vi "Read_from_Config_File.vi"(11 "Error In":errorcluster) -> (4 "Debug":bool, 15 "Error Out":errorcluster)   [LabVIEW 2026, in "Core.lvlib"]
doc: "Reads application settings from the configuration file and returns the configured status."
uses:
  Core.lvlib
  <vilib>/Utility/config.llb/Read Key (Boolean).vi
  <vilib>/Utility/config.llb/NI_LVConfig.lvlib
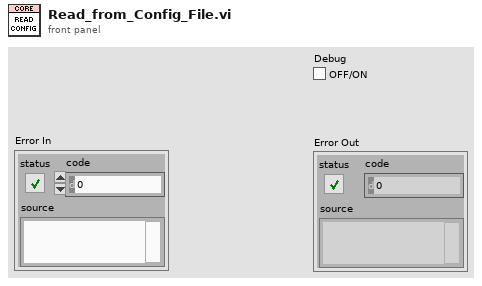
[diagram p1: front panel]
types:
  T1 = typedef "NI_LVConfig.lvlib/Config Data RefNum.ctl" = refnum<k1>
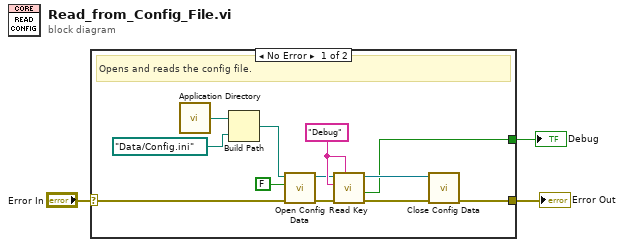
[diagram p0: block diagram]
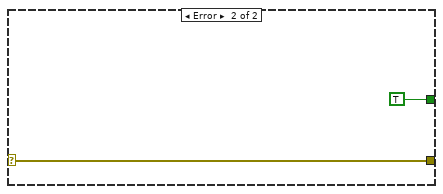
[diagram p2: hidden frame]
diagram:
  n1 = case shown="No Error" "Error In" {
    selector: "Error In" -> [w9 w16]
    tunnel: [w15 w16] -> w3
    tunnel: [w12 TRUE] -> w2
    frame No Error {
      w11 = "Debug" ("section")
      # "Opens and reads the config file."
      n2 = call <vilib>:"Application Directory.vi"() -> ("Application Directory"=w5:path)
      n3 = Build Path(base path=w5, name or relative path=path "Data/Config.ini") -> (appended path=w7:path)
      n4 = call <vilib>:"Open Config Data.vi"("error in (no error)"=w9, "create file if necessary (T)"=FALSE, "configuration file path"=w7) -> ("error out"=w10:errorcluster, "refnum"=w4:T1)  [unwired: 6 in, 1 out]
      n5 = call-poly <vilib>:"Read Key.vi"("section"=w11, "error in (no error)"=w10, "key"=w11, "refnum"=w4) -> ("error out"=w14:errorcluster, "value"=w12:bool, "refnum out"=w13:T1)  [unwired: 4 in, 1 out]
      n6 = call <vilib>:"Close Config Data.vi"("error in (no error)"=w14, "refnum"=w13) -> ("error out"=w15:errorcluster)  [unwired: 8 in, 1 out]
    }
    frame Error {
    }
  }
  "Error Out" <- w3
  "Debug" <- w2
